vi "UMLEditor Main.vi"(1 "StartProject":string, 3 "StartTarget":string) -> ()   [LabVIEW 2020] (continued)
        n1589 = property class="Project"(reference=w4295) -> (reference out=w4292:refnum<vi>, error out=w4293:errorcluster, "Path"=w4291:path)  [unwired: 1 in]
        n1590 = call <resource>:"GetRelativePathOption.vi"() -> ("UseProjectFolderAsBasePath"=w4294:bool)  [unwired: 1 in, 18 out]
        n1591 = Strip Path(path=w4291) -> (stripped path=w4288:path)  [unwired: 1 out]
        n1592 = Close Reference(reference=w4292, error in (no error)=w4293) -> (error out=w4287:errorcluster)
        n1593 = call <resource>:"File_ApplicationPaths.vi"("PathName"=UMLEditor_StoredPathes."LastSearchPath" ("UMLPathes"), "Path In"=w4288, "Method (Get Path)"=File_StoredPathesActions."Set Path") -> ()  [unwired: 1 in, 16 out]
        n1594 = case shown="True" w4294 {
          tunnel: w4288 -> [_ w4305]
          tunnel: w4287 -> [_ _]
          frame False {
          }
          frame True {
            n1595 = call <resource>:"File_ApplicationPaths.vi"("PathName"=UMLEditor_StoredPathes."ClassBasePath" ("UMLPathes"), "Path In"=w4305, "Method (Get Path)"=File_StoredPathesActions."Set Path") -> ()  [unwired: 1 in, 16 out]
          }
        }
      }
      frame "ClassReversedEngineering".."StateReversedEngineering" {
        n1596 = case shown="\"ClassReversedEngineering\", Default" w4310 {
          tunnel: w4317 -> [w4331 w4367 w4387]
          tunnel: [w4320 w4366 w4382] -> w4315
          tunnel: [w4323 w4365 w4387] -> w4314
          tunnel: [w4319 w4364 w4381] -> w4312
          tunnel: w4309 -> [w4318 w4361 w4383]
          tunnel: [w4318 w4362 w4383] -> w4308
          frame "StateReversedEngineering" {
            (unwired) T49."existing file" ("select mode (2)")
            n1597 = Unbundle By Name(w4318) -> ("grid"=w4321:refnum<class "Grid.lvclass">, "graphics"=w4322:refnum<class "Graphics.lvclass">)
            n1598 = File Dialog(4:"VIs" ("pattern label"), 6:"*.vi" ("pattern"), 7:"Select VI(containing a state machine) for analysing" ("prompt")) -> (1:w4327:bool, 3:w4326:path)  [unwired: 1 in, 5 out]
            n1599 = Bundle By Name(cluster=T29 {"VI-Path"=path "", "ShowOption"=enum."Show Relative Path"} ("StateDiagramData"), "VI-Path"=w4326) -> (w4324:T29)
            n1600 = case shown="False" w4327 {
              selector: w4327 -> [_ w4348]
              tunnel: w4331 -> [w4342 w4347]
              tunnel: w4324 -> [w4341 _]
              tunnel: [w4334 w4347] -> w4323
              tunnel: w4322 -> [w4338 _]
              tunnel: w4321 -> [w4337 _]
              tunnel: [w4333 w4348] -> w4320
              tunnel: [w4332 _] -> w4319
              frame False {
                n1601 = call <resource>:"StateDiagramGraph_Create.vi"("StateDiagramData"=w4341, "error in (no error)"=w4342) -> ("reference out"=w4340:refnum<class "StateDiagramGraph.lvclass">, "error out"=w4339:errorcluster)  [unwired: 1 in, 15 out]
                n1602 = call-dynamic "HandleRightClickMenuOption.vi"("reference"=w4340, "MenuOption"="Create New Diagram", "graphics"=w4338, "grid"=w4337, "error in (no error)"=w4339) -> ("reference out"=w4332:refnum<class "StateDiagramGraph.lvclass">, "Cancel"=w4333:bool, "error out"=w4335:errorcluster)  [unwired: 12 in]
                n1603 = case shown="False" w4333 {
                  tunnel: w4332 -> [_ w4346]
                  tunnel: w4335 -> [w4343 w4345]
                  tunnel: [w4343 w4344] -> w4334
                  frame False {
                  }
                  frame True {
                    n1604 = call-dynamic "Destroy.vi"("reference"=w4346, "error in (no error)"=w4345) -> ("error out"=w4344:errorcluster)  [unwired: 17 in]
                  }
                }
              }
              frame True {
              }
            }
          }
          frame "ClassReversedEngineering", Default {
            n1605 = Unbundle By Name(w4361) -> ("XMI_Import"=w4349:bool, "Action"=w4358:string)
            n1606 = String To Path(string=w4358) -> (path=w4351:path)
            n1607 = File/Directory Info(path=w4351) -> (size=w4357:i64)  [unwired: 1 in, 6 out]
            n1608 = call <vilib>:"Librarian Get Info.vi"("path"=w4351) -> ("file information"=w4355:T55)  [unwired: 1 in, 9 out]
            n1609 = Unbundle By Name(w4355) -> ("size"=w4354:i32)
            n1610 = Greater Than 0?(x=w4357) -> (x > 0?=w4356:bool)
            n1611 = Greater Than 0?(x=w4354) -> (x > 0?=w4353:bool)
            n1612 = Equal?(x=w4358, y="WholeProject") -> (x = y?=w4359:bool)
            n1613 = Or(x=w4356, y=w4353) -> (x .or. y?=w4352:bool)
            n1614 = case shown="False" w4352 {
              tunnel: w4367 -> [w4373 w4379]
              tunnel: [w4372 w4378] -> w4366
              tunnel: [w4371 w4377] -> w4365
              tunnel: [w4370 w4376] -> w4364
              tunnel: w4359 -> [w4369 _]
              tunnel: w4351 -> [_ w4375]
              tunnel: w4349 -> [w4368 w4374]
              frame False {
                n1615 = call <resource>:"UMLEditor reversedEngineering.vi"("AddProjectClasses"=w4369, "XMI Import"=w4368, "error in (no error)"=w4373) -> ("cancel"=w4372:bool, "newCLassDiagram"=w4370:refnum<class "Graph.lvclass">, "error out"=w4371:errorcluster)  [unwired: 1 in, 13 out]
              }
              frame True {
                n1616 = call <resource>:"UMLEditor reversedEngineering.vi"("ClassToAnalyse/XMI File To Read"=w4375, "XMI Import"=w4374, "error in (no error)"=w4379) -> ("cancel"=w4378:bool, "newCLassDiagram"=w4376:refnum<class "Graph.lvclass">, "error out"=w4377:errorcluster)  [unwired: 1 in, 13 out]
              }
            }
            n1617 = Bundle By Name(cluster=w4361, "Action"="", "XMI_Import"=FALSE) -> (w4362:T5)
          }
          frame "PlugInReverseEngineering" {
            n1618 = call <resource>:"File_ApplicationPaths.vi"("PathName"=UMLEditor_StoredPathes."RevPlugInPath" ("UMLPathes")) -> ("Path Out"=w4384:path)  [unwired: 3 in, 15 out]
            n1619 = Open VI Reference(type specifier VI Refnum (for type only)=refnum<vi> refnum, vi path=w4384, error in (no error)=w4387) -> (vi reference=w4391:refnum<vi>, error out=w4390:errorcluster)  [unwired: 3 out]
            n1620 = call-by-ref "?"(reference=w4391, error in=w4390) -> (reference out=w4389:refnum<vi>, error out=w4388:errorcluster, "reference"=w4381:refnum<class "Graph.lvclass">, "cancelled"=w4382:bool, "diagramType"=w4380:T56)  [unwired: 8 in, 1 out]
            n1621 = Close Reference(reference=w4389, error in (no error)=w4388) -> (error out=w4386:errorcluster)
            n1622 = Format Into String(w4380) -> ()  [unwired: 3 in, 2 out]
            n1623 = call <vilib>:"Simple Error Handler.vi"("error in (no error)"=w4386) -> ()  [unwired: 1 in, 8 out]
          }
        }
        n1624 = case shown="False" w4315 {
          tunnel: w4314 -> [w4406 w4430]
          tunnel: [w4412 w4430] -> w4316
          tunnel: [w4410 w4428] -> w4313
          tunnel: w4312 -> [w4407 _]
          tunnel: [UMLEditor_statesType."Repaint" ("state") UMLEditor_statesType."Idle" ("state")] -> w4311
          tunnel: w4308 -> [w4396 w4428]
          frame False {
            n1625 = Unbundle By Name(w4396) -> ("diagrams"=w4422:T8[])
            n1626 = Unbundle By Name(w4396) -> ("grid"=w4403:refnum<class "Grid.lvclass">, "graphics"=w4404:refnum<class "Graphics.lvclass">)
            n1627 = for {
              tunnel: w4422 -> [w4427] mode=indexing
              tunnel: "Untitled %d" -> [w4425]
              tunnel: [w4424] -> w4420 mode=indexing
              n1628 = Unbundle By Name(w4427) -> ("name"=w4426:string)
              n1629 = Scan From String(format string=w4425, input string=w4426) -> (output 1=w4424:i32)  [unwired: 2 in, 4 out]
            }
            n1630 = Array Max & Min(array=w4420) -> (max value=w4419:i32)  [unwired: 3 out]
            n1631 = call-dynamic "draw.vi"("reference"=w4407, "graphics"=w4404, "grid"=w4403, "error in (no error)"=w4406, "SelectedNodes"=refnum<class "AbstractNode.lvclass">[] [], "HideOverLays(False)"=FALSE) -> ("NodesBounds"=w4402:T10, "error out"=w4405:errorcluster)  [unwired: 10 in, 2 out]
            n1632 = Increment(x=w4419) -> (x+1=w4417:i32)
            n1633 = Bundle By Name(cluster=w4396, "NodesBounds"=w4402) -> (w4399:T5)
            n1634 = Format Into String(format string="Untitled %d", w4417) -> (resulting string=w4408:string)  [unwired: 2 in, 1 out]
            n1635 = property on="Diagram" class="Ring (strict)"("Tip Strip"=w4408) -> ()  [unwired: 2 in, 2 out]
            n1636 = Unbundle By Name(w4399) -> ("menu"=w4398:refnum<k9>)
            n1637 = call <resource>:"UMLEditor addDiagram.vi"("graph"=w4407, "name"=w4408, "saveDir"=path "", "unsaved(False)"=TRUE, "error in (no error)"=w4405, "localVariablesIn"=w4399) -> ("localVariablesOut"=w4397:T5, "error out"=w4415:errorcluster)  [unwired: 1 in, 11 out]
            n1638 = property on="GraphButtons" class="RadioBtnsControl (strict)"("Disabled"=u8 0) -> ()  [unwired: 2 in, 2 out]
            n1639 = call <resource>:"UMLEditor menuUpdates.vi"("menu"=w4398, "menuAction"=UMLEditor_MenuActionType."EnableSave", "error in (no error)"=w4415) -> ("error out"=w4411:errorcluster)  [unwired: 3 in, 13 out]
            n1640 = local write "Diagram"(0) -> ()
            n1641 = property on="Picture" class="Pict"("Visible"=TRUE) -> ()  [unwired: 2 in, 2 out]
            n1642 = call <resource>:"UMLEditor setDiagramInfo.vi"("error in (no error)"=w4411, "localVariablesIn"=w4397, "action"=enum16{"Name/Dir", "Unsaved", "Saved"}."Unsaved") -> ("localVariablesOut"=w4410:T5, "error out"=w4412:errorcluster)  [unwired: 2 in, 13 out]
          }
          frame True {
          }
        }
      }
      frame "PanAndRepaint" {
        n1643 = Unbundle By Name(w4450) -> ("graphics"=w4449:refnum<class "Graphics.lvclass">, "SelectedNodes"=w4448:refnum<class "AbstractNode.lvclass">[])
        n1644 = Index Array(array=w4448) -> (element=w4447:refnum<class "AbstractNode.lvclass">)  [unwired: 1 in]
        n1645 = To More Specific Class(target class=refnum<class "RectangularNode.lvclass"> refnum ("reference"), reference=w4447, error in=w4445) -> (specific class reference=w4444:refnum<class "RectangularNode.lvclass">, error out=w4443:errorcluster)
        n1646 = call <resource>:"getScreenBounds.vi"("reference"=w4449) -> ("bounds"=w4438:T10)  [unwired: 1 in, 17 out]
        n1647 = call-dynamic "getBounds.vi"("reference"=w4444, "error in (no error)"=w4443) -> ("bounds"=w4432:T10, "error out"=w4434:errorcluster)  [unwired: 15 in, 1 out]
        n1648 = Unbundle By Name(w4438) -> ("width"=w4433:dbl, "height"=w4431:dbl)
        n1649 = property on="Picture" class="Pict"() -> ("Origin:Left"=w4440:i16, "Origin:Top"=w4439:i16)  [unwired: 2 in, 2 out]
        n1650 = Unbundle By Name(w4432) -> ("x"=w4442:dbl, "y"=w4441:dbl)
        n1651 = In Range and Coerce(upper limit=w4433, x=w4442, lower limit=w4440) -> (In Range?=w4437:bool)  [unwired: 1 out]
        n1652 = In Range and Coerce(upper limit=w4431, x=w4441, lower limit=w4439) -> (In Range?=w4436:bool)  [unwired: 1 out]
        n1653 = And(x=w4437, y=w4436) -> (x .and. y?=w4435:bool)
        n1654 = case shown="False" w4435 {
          tunnel: w4433 -> [w4465 _]
          tunnel: w4432 -> [w4463 _]
          tunnel: w4431 -> [w4458 _]
          frame False {
            w4452 = 0.0 ("y")
            n1655 = call <resource>:"Rectangel GetRectInfo.vi"("bounds"=w4463) -> ("centerX"=w4462:dbl, "centerY"=w4460:dbl)  [unwired: 14 in, 3 out]
            n1656 = Divide(x=w4465, y=2.0) -> (x/y=w4461:dbl)
            n1657 = Divide(x=w4458, y=2.0) -> (x/y=w4457:dbl)
            n1658 = Subtract(x=w4462, y=w4461) -> (x-y=w4456:dbl)
            n1659 = Subtract(x=w4460, y=w4457) -> (x-y=w4454:dbl)
            n1660 = Max & Min(x=w4456, y=w4452) -> (max(x,y)=w4455:dbl)  [unwired: 1 out]
            n1661 = Max & Min(x=w4454, y=w4452) -> (max(x,y)=w4453:dbl)  [unwired: 1 out]
            n1662 = property on="Picture" class="Pict"("Origin:Left"=w4455, "Origin:Top"=w4453) -> ()  [unwired: 2 in, 2 out]
          }
          frame True {
          }
        }
      }
      frame "Repaint" {
        n1663 = Unbundle By Name(w4474) -> ("selected"=w4486:T7)
        n1664 = call <resource>:"UMLEditor getDiagramInfo.vi"("localVariables"=w4474, "error in (no error)"=w4484) -> ("graph"=w4471:refnum<class "Graph.lvclass">, "diagramType"=w4478:T27, "error out"=w4479:errorcluster)  [unwired: 15 out]
        n1665 = case shown="\"Node\"" w4486 {
          tunnel: [w4499 UMLEditor_MenuActionType."enablePropDel" ("menuAction") UMLEditor_MenuActionType."enablePropDel" ("menuAction")] -> w4485
          tunnel: w4478 -> [w4498 _ _]
          tunnel: [UMLEditor_MenuActionType."DisableCopy" ("menuAction") UMLEditor_MenuActionType."EnableCopy" ("menuAction") UMLEditor_MenuActionType."DisableCopy" ("menuAction")] -> w4468
          frame "None", Default {
            n1666 = case shown="Default" w4498 {
              tunnel: [UMLEditor_MenuActionType."enablePropDisDel" ("menuAction") UMLEditor_MenuActionType."disablePropDel" ("menuAction")] -> w4499
              frame "StateDiagramGraph" {
              }
              frame Default {
              }
            }
          }
          frame "Node" {
          }
          frame "Edge" {
          }
        }
        n1667 = Unbundle By Name(w4474) -> ("menu"=w4469:refnum<k9>)
        n1668 = Empty String/Path?(string/path=w4478) -> (empty?=w4483:bool)
        n1669 = call <resource>:"UMLEditor ToolsMenuUpdates.vi"("menu"=w4469, "Graph"=w4471, "error in (no error)"=w4479) -> ("error out"=w4467:errorcluster)  [unwired: 3 in, 13 out]
        n1670 = disable-structure shown="Enabled" {
          disable-tunnel: w4469 -> [w4495 _]
          disable-tunnel: w4468 -> [w4494 _]
          disable-tunnel: w4467 -> [w4493 w4496]
          disable-tunnel: [w4492 w4496] -> w4466
          frame Disabled {
            n1671 = call <resource>:"UMLEditor menuUpdates.vi"("menu"=w4495, "menuAction"=w4494, "error in (no error)"=w4493) -> ("error out"=w4492:errorcluster)  [unwired: 3 in, 13 out]
          }
          frame Enabled {
          }
        }
        n1672 = call <resource>:"UMLEditor menuUpdates.vi"("menu"=w4469, "menuAction"=w4485, "error in (no error)"=w4466) -> ("error out"=w4487:errorcluster)  [unwired: 3 in, 13 out]
        n1673 = call <resource>:"UMLEditor updateDiagramsInfo.vi"("localVariables"=w4474, "error in (no error)"=w4487) -> ("diagramNames"=w4491:string[], "index"=w4477:i32, "currentIsUnsaved"=w4473:bool, "notSavedBefore"=w4488:bool, "error out"=w4472:errorcluster)  [unwired: 13 out]
        n1674 = property on="Diagram" class="Ring (strict)"() -> ("Strings []"=w4490:string[])  [unwired: 2 in, 2 out]
        n1675 = feedback #6() -> (w4470:i32)  [unwired: 1 in]
        n1676 = feedback-in #6(w4477) -> ()
        n1677 = Not Equal?(x=w4470, y=w4477) -> (x != y?=w4475:bool)
        n1678 = Not Equal?(x=w4491, y=w4490) -> (x != y?=w4489:bool)
        n1679 = Or(x=w4475, y=w4489) -> (x .or. y?=w4476:bool)
        n1680 = case shown="True" w4476 {
          tunnel: w4491 -> [_ w4510]
          tunnel: w4477 -> [_ w4508]
          tunnel: w4473 -> [_ w4507]
          tunnel: w4488 -> [_ w4509]
          tunnel: w4469 -> [_ w4506]
          frame False {
          }
          frame True {
            (unwired) u16 0 items=["Class diagram: Untitled 1 *"] ("Diagram")
            n1681 = Compound Arithmetic op=AND(w4507, invert w4509) -> ()  [unwired: 1 out]
            n1682 = property on="Diagram" class="Ring (strict)"("Strings []"=w4510) -> ()  [unwired: 2 in, 2 out]
            n1683 = local write "Diagram"(w4508) -> ()
            n1684 = case shown="False" w4507 {
              tunnel: w4506 -> [w4511 w4513]
              frame True {
                n1685 = call <resource>:"UMLEditor menuUpdates.vi"("menu"=w4511, "menuAction"=UMLEditor_MenuActionType."EnableSave") -> ()  [unwired: 4 in, 14 out]
              }
              frame False {
                n1686 = call <resource>:"UMLEditor menuUpdates.vi"("menu"=w4513, "menuAction"=UMLEditor_MenuActionType."DiableSave") -> ()  [unwired: 4 in, 14 out]
              }
            }
          }
        }
        n1687 = Select(t=UMLEditor_statesType."Idle", s=w4483, f=UMLEditor_statesType."PaintComponent" ("state")) -> (s? t:f=w4481:T6)
      }
      frame "PaintComponent" {
        n1688 = Unbundle By Name(w4528) -> ("menu"=w4527:refnum<k9>)
        n1689 = Unbundle By Name(w4528) -> ("selected"=w4537:T7, "selectedEdge"=w4547:refnum<class "AbstractEdge.lvclass">, "SelectedNodes"=w4522:refnum<class "AbstractNode.lvclass">[], "ObjectHotspots"=w4521:T15[], "NodesBounds"=w4535:T10)
        n1690 = Unbundle By Name(w4528) -> ("newSelected"=w4544:bool, "zoom"=w4551:dbl, "grid"=w4545:refnum<class "Grid.lvclass">, "offset"=w4538:T9, "graphics"=w4541:refnum<class "Graphics.lvclass">, "hideGrid"=w4550:bool)  [unwired: 1 out]
        n1691 = Unbundle By Name(w4528) -> ("butDwn"=w4531:bool)
        n1692 = Unbundle By Name(w4528) -> ("ResizePanelInProgress"=w4532:bool)
        n1693 = call <resource>:"UMLEditor getDiagramInfo.vi"("localVariables"=w4528, "error in (no error)"=w4549) -> ("graph"=w4529:refnum<class "Graph.lvclass">, "error out"=w4539:errorcluster)  [unwired: 16 out]
        n1694 = case shown="False" w4544 {
          tunnel: w4551 -> [w4567 _]
          tunnel: w4550 -> [w4568 _]
          tunnel: w4529 -> [w4583 w4615]
          tunnel: [w4582 w4615] -> w4548
          tunnel: [w4581 w4616] -> w4530
          tunnel: w4539 -> [w4580 w4616]
          tunnel: w4541 -> [w4579 _]
          tunnel: w4545 -> [w4578 _]
          tunnel: w4540 -> [_ _]
          tunnel: w4538 -> [w4577 _]
          tunnel: [w4570 w4614] -> w4536
          tunnel: w4535 -> [w4571 w4614]
          tunnel: w4522 -> [w4563 _]
          tunnel: [w4562 w4611] -> w4519
          tunnel: w4521 -> [_ w4613]
          frame False {
            n1695 = call <resource>:"resetPicture.vi"("reference"=w4579, "error in (no error)"=w4580) -> ("reference out"=w4576:refnum<class "Graphics.lvclass">, "error out"=w4575:errorcluster)  [unwired: 16 out]
            n1696 = call <resource>:"getScreenBounds.vi"("reference"=w4576, "error in (no error)"=w4575) -> ("reference out"=w4574:refnum<class "Graphics.lvclass">, "bounds"=w4572:T10, "ZoomChanged"=w4564:bool, "error out"=w4573:errorcluster)  [unwired: 14 out]
            n1697 = Less?(x=w4567, y=0.5) -> (x < y?=w4565:bool)
            n1698 = Or(x=w4565, y=w4568) -> (x .or. y?=w4569:bool)
            n1699 = case shown="False" w4569 {
              tunnel: w4578 -> [w4609 _]
              tunnel: w4567 -> [_ _]
              tunnel: [w4608 w4610] -> w4584
              tunnel: w4577 -> [_ _]
              tunnel: w4574 -> [w4607 _]
              tunnel: w4573 -> [w4606 w4610]
              tunnel: w4572 -> [w4601 _]
              tunnel: w4571 -> [w4605 _]
              tunnel: w4564 -> [w4590 _]
              frame False {
                w4585 = 500
                w4603 = 50
                w4600 = 0.0 ("x")
                n1700 = Unbundle By Name(w4605) -> ("width"=w4604:dbl, "height"=w4602:dbl)
                n1701 = Unbundle By Name(w4601) -> ("width"=w4599:dbl, "height"=w4598:dbl)
                n1702 = property on="Picture" class="Pict"() -> ("Origin:Left"=w4593:i16, "Origin:Top"=w4592:i16)  [unwired: 2 in, 2 out]
                n1703 = Add(x=w4603, y=w4602) -> (x+y=w4594:dbl)
                n1704 = Add(x=w4603, y=w4604) -> (x+y=w4597:dbl)
                n1705 = Add(x=w4593, y=w4599) -> (x+y=w4596:dbl)
                n1706 = Add(x=w4592, y=w4598) -> (x+y=w4595:dbl)
                n1707 = Max & Min(x=w4597, y=w4596) -> (max(x,y)=w4589:dbl)  [unwired: 1 out]
                n1708 = Max & Min(x=w4594, y=w4595) -> (max(x,y)=w4587:dbl)  [unwired: 1 out]
                n1709 = Add(x=w4585, y=w4587) -> (x+y=w4586:dbl)
                n1710 = Add(x=w4585, y=w4589) -> (x+y=w4588:dbl)
                n1711 = Bundle(cluster=w4601, "x"=w4600, "y"=w4600, "width"=w4588, "height"=w4586) -> (w4591:T10)
                n1712 = call-dynamic "draw.vi"("reference"=w4609, "graphics"=w4607, "bounds"=w4591, "ForceRedrawGrid"=w4590, "error in (no error)"=w4606) -> ("error out"=w4608:errorcluster)  [unwired: 13 in, 1 out]
              }
              frame True {
              }
            }
            n1713 = call-dynamic "draw.vi"("reference"=w4583, "graphics"=w4579, "grid"=w4578, "error in (no error)"=w4584, "SelectedNodes"=w4563, "HideOverLays(False)"=FALSE) -> ("reference out"=w4582:refnum<class "Graph.lvclass">, "NodesBounds"=w4570:T10, "HotSpots"=w4562:T15[], "error out"=w4581:errorcluster)  [unwired: 10 in]
          }
          frame True {
            n1714 = for {
              tunnel: w4613 -> [w4618] mode=indexing
              shift-right: [w4617] -> w4611
              shift-left: T15[] [] -> [w4619]
              n1715 = Unbundle By Name(w4618) -> ("Function"=w4620:T16)
              n1716 = case shown="\"Expand\", \"Collaps\"" w4620 {
                tunnel: w4619 -> [w4621 w4624]
                tunnel: w4618 -> [_ w4623]
                tunnel: [w4621 w4622] -> w4617
                frame Default {
                }
                frame "Expand", "Collaps" {
                  n1717 = Build Array (concatenate)(w4624, w4623) -> (w4622:T15[])
                }
              }
            }
          }
        }
        n1718 = Compound Arithmetic op=AND(invert w4531, invert w4532) -> (w4526:bool)
        n1719 = call <resource>:"UMLEditor_GraphMemory.vi"("GraphIn"=w4529) -> ()  [unwired: 1 in, 18 out]
        n1720 = call <resource>:"updateScreen.vi"("reference"=w4541, "error in (no error)"=w4530) -> ("reference out"=w4525:refnum<class "Graphics.lvclass">, "picture"=w4515:picture, "error out"=w4542:errorcluster)  [unwired: 15 out]
        n1721 = case shown="True" w4526 {
          tunnel: w4530 -> [w4555 w4560]
          tunnel: [w4555 w4559] -> _
          tunnel: w4529 -> [_ w4558]
          tunnel: w4527 -> [_ w4556]
          frame False {
          }
          frame True {
            n1722 = call <resource>:"UndoEngine.vi"("Reference In"=w4558, "Action"=enum16{"TakeSnapshot", "Undo", "Redo"}."TakeSnapshot", "error in (no error)"=w4560, "menu"=w4556) -> ("error out"=w4559:errorcluster)  [unwired: 4 in, 11 out]
          }
        }
        n1723 = case shown="\"Edge\"" w4537 {
          tunnel: [w4628 w4637 w4676] -> w4518
          tunnel: w4548 -> [_ w4640 w4682]
          tunnel: w4542 -> [w4628 w4639 w4681]
          tunnel: w4547 -> [_ w4633 _]
          tunnel: [TRUE w4632 w4678] -> w4533
          tunnel: w4541 -> [_ w4636 w4675]
          tunnel: w4522 -> [_ _ w4680]
          tunnel: w4525 -> [_ w4631 w4672]
          tunnel: [w4626 w4630 w4673] -> w4520
          tunnel: w4519 -> [w4626 w4630 w4671]
          tunnel: w4515 -> [w4625 w4629 w4668]
          frame "None", Default {
            n1724 = local write "Picture"(w4625) -> ()
          }
          frame "Edge" {
            n1725 = call-dynamic "getEdges.vi"("reference"=w4640, "error in (no error)"=w4639) -> ("edges"=w4638:refnum<class "AbstractEdge.lvclass">[], "error out"=w4635:errorcluster)  [unwired: 15 in, 1 out]
            n1726 = Search 1D Array(1D array=w4638, element=w4633) -> (index of element=w4634:i32)  [unwired: 1 in]
            n1727 = case shown="0, Default" w4634 {
              tunnel: [w4655 w4667] -> w4637
              tunnel: w4636 -> [w4654 _]
              tunnel: w4635 -> [w4653 w4667]
              tunnel: w4633 -> [w4643 _]
              tunnel: w4631 -> [w4641 _]
              tunnel: w4629 -> [_ w4666]
              frame 0, Default {
                n1728 = To More Specific Class(target class=refnum<class "GeneralPathEdge.lvclass"> refnum ("reference out"), reference=w4643) -> (specific class reference=w4642:refnum<class "GeneralPathEdge.lvclass">, error out=w4644:errorcluster)  [unwired: 1 in]
                n1729 = case shown="No Error" w4644 {
                  tunnel: w4653 -> [w4660 w4665]
                  tunnel: [w4656 w4664] -> w4652
                  tunnel: [w4657 w4663] -> w4651
                  tunnel: [w4658 w4662] -> w4649
                  tunnel: w4643 -> [_ w4661]
                  tunnel: w4642 -> [w4659 _]
                  frame No Error {
                    n1730 = call-dynamic "getPath.vi"("reference"=w4659, "error in (no error)"=w4660) -> ("reference out"=w4658:refnum<class "GeneralPathEdge.lvclass">, "points"=w4656:T9[], "error out"=w4657:errorcluster)  [unwired: 15 in]
                  }
                  frame Error {
                    n1731 = call-dynamic "getConnectionPoints.vi"("reference"=w4661, "error in (no error)"=w4665) -> ("reference out"=w4662:refnum<class "AbstractEdge.lvclass">, "connectionPoints"=w4664:T9[], "error out"=w4663:errorcluster)  [unwired: 15 in]
                  }
                }
                n1732 = call-dynamic "GetTextPositions.vi"("reference"=w4649, "GraphicsRef"=w4641, "error in (no error)"=w4651) -> ("connectionPoints"=w4647:T9[], "error out"=w4650:errorcluster)  [unwired: 14 in, 1 out]
                n1733 = Build Array (concatenate)(w4652, w4647) -> (w4648:T9[])
                n1734 = call <resource>:"UMLEditor drawGrabbers.vi"("graphics"=w4654, "points"=w4648, "error in (no error)"=w4650) -> ("picture"=w4646:picture, "error out"=w4655:errorcluster)  [unwired: 15 out]
                n1735 = local write "Picture"(w4646) -> ()
              }
              frame -1 {
                "Picture" <- w4666
              }
            }
            n1736 = Less Than 0?(x=w4634) -> (x < 0?=w4632:bool)
          }
          frame "Node" {
            n1737 = Array Size(array=w4680) -> (size(s)=w4679:i32)
            n1738 = for {
              tunnel: w4682 -> [w4700]
              tunnel: w4680 -> [w4696] mode=indexing
              shift-right: [w4695] -> w4677
              shift-left: w4681 -> [_]
              shift-right: [w4693] -> w4670
              shift-left: T9[] [] -> [w4694]
              shift-right: [w4692] -> w4673
              shift-left: w4671 -> [w4691]
              tunnel: w4672 -> [w4690]
              n1739 = call-dynamic "getNodes.vi"("reference"=w4700) -> ("nodes"=w4699:refnum<class "AbstractNode.lvclass">[], "error out"=w4698:errorcluster)  [unwired: 16 in, 1 out]
              n1740 = Search 1D Array(1D array=w4699, element=w4696) -> (index of element=w4697:i32)  [unwired: 1 in]
              n1741 = case shown="0, Default" w4697 {
                tunnel: [w4701 w4712] -> w4695
                tunnel: w4698 -> [w4708 w4712]
                tunnel: w4696 -> [w4703 _]
                tunnel: w4694 -> [w4709 w4711]
                tunnel: [w4707 w4711] -> w4693
                tunnel: [w4706 w4710] -> w4692
                tunnel: w4691 -> [w4705 w4710]
                tunnel: w4690 -> [_ _]
                frame 0, Default {
                  n1742 = call-dynamic "GetGrabberPositions.vi"("reference"=w4703, "error in (no error)"=w4708) -> ("GrabberPositions"=w4704:T9[], "HotSpots"=w4702:T15[], "error out"=w4701:errorcluster)  [unwired: 14 in, 1 out]
                  n1743 = Build Array (concatenate)(w4705, w4702) -> (w4706:T15[])
                  n1744 = Build Array (concatenate)(w4709, w4704) -> (w4707:T9[])
                }
                frame -1 {
                }
              }
            }
            n1745 = Less Or Equal To 0?(x=w4679) -> (x <= 0?=w4678:bool)
            n1746 = Empty Array?(array=w4670) -> (empty?=w4669:bool)
            n1747 = case shown="False" w4669 {
              tunnel: w4677 -> [w4687 w4689]
              tunnel: [w4686 w4689] -> w4676
              tunnel: w4675 -> [w4685 _]
              tunnel: w4670 -> [w4684 _]
              tunnel: w4668 -> [_ w4688]
              frame False {
                n1748 = call <resource>:"UMLEditor drawGrabbers.vi"("graphics"=w4685, "points"=w4684, "error in (no error)"=w4687) -> ("picture"=w4683:picture, "error out"=w4686:errorcluster)  [unwired: 15 out]
                n1749 = local write "Picture"(w4683) -> ()
              }
              frame True {
                n1750 = local write "Picture"(w4688) -> ()
              }
            }
          }
        }
        n1751 = Bundle By Name(cluster=w4528, "newSelected"=FALSE, "NodesBounds"=w4536) -> (w4534:T5)
        n1752 = case shown="True" w4533 {
          tunnel: [w4713 w4715] -> w4523
          tunnel: w4534 -> [w4713 w4716]
          frame False {
          }
          frame True {
            n1753 = Bundle By Name(cluster=w4716, "selected"=UMLEditor_tooltype."None" ("selcted")) -> (w4715:T5)
          }
        }
        n1754 = Tick Count (ms)() -> (millisecond timer value=w4516:u32)
        n1755 = case shown="True" w4517 {
          tunnel: w4518 -> [_ _]
          tunnel: w4516 -> [_ w4552]
          frame False {
          }
          frame True {
            n1756 = Tick Count (ms)() -> (millisecond timer value=w4554:u32)
            n1757 = Subtract(x=w4554, y=w4552) -> (x-y=→"Time":u32)
          }
        }
        n1758 = Bundle By Name(cluster=w4523, "ObjectHotspots"=w4520) -> (w4524:T5)
      }
      frame "AutoPlace" {
        n1759 = call <resource>:"ArrangeNodes Main.vi"("localVariablesOut"=w4719) -> ("Cancel"=w4717:bool)  [unwired: 1 in, 17 out]
        n1760 = case shown="False" w4717 {
          tunnel: w4721 -> [w4724 w4730]
          tunnel: [w4724 w4729] -> w4720
          tunnel: [w4723 w4726] -> w4718
          tunnel: w4719 -> [w4723 w4728]
          frame True {
          }
          frame False {
            n1761 = call <resource>:"UMLEditor setDiagramInfo.vi"("error in (no error)"=w4730, "localVariablesIn"=w4728, "action"=enum16{"Name/Dir", "Unsaved", "Saved"}."Unsaved") -> ("localVariablesOut"=w4727:T5, "error out"=w4729:errorcluster)  [unwired: 2 in, 13 out]
            n1762 = Bundle By Name(cluster=w4727, "modified"=TRUE) -> (w4726:T5)
          }
        }
      }
      frame "ExecuteCommand" {
        n1763 = Unbundle By Name(w4735) -> ("FlattenCommandSettings.Command"=w4743:T13, "FlattenCommandSettings.CommandData"=w4737:variant, "selected"=w4742:T7, "selectedEdge"=w4732:refnum<class "AbstractEdge.lvclass">, "SelectedNodes"=w4739:refnum<class "AbstractNode.lvclass">[])
        n1764 = Unbundle By Name(w4735) -> ("graphics"=w4734:refnum<class "Graphics.lvclass">, "grid"=w4733:refnum<class "Grid.lvclass">)
        n1765 = call <resource>:"UMLEditor getDiagramInfo.vi"("localVariables"=w4735, "error in (no error)"=w4741) -> ("graph"=w4736:refnum<class "Graph.lvclass">, "error out"=w4740:errorcluster)  [unwired: 16 out]
        n1766 = case shown="\"SyncCodeFromUML\"" w4743 {
          tunnel: [w4756 w4832 UMLEditor_statesType."Idle" ("state") UMLEditor_statesType."Idle" ("state") UMLEditor_statesType."CreateScript" ("state") UMLEditor_statesType."Idle" ("state") UMLEditor_statesType."Idle" ("state") w5042 UMLEditor_statesType."Idle" ("state")] -> w4745
          tunnel: w4740 -> [w4755 w4839 w4863 w4868 w4893 w4899 w4916 w5060 w5086]
          tunnel: [w4752 w4844 w4863 w4868 w4893 w4898 w4914 w5060 w5085] -> w4744
          tunnel: w4742 -> [w4754 w4837 _ _ _ _ _ _ _]
          tunnel: w4739 -> [w4753 w4835 _ _ _ _ _ w5061 w5083]
          tunnel: w4735 -> [w4751 w4843 w4865 w4881 w4891 w4908 w4921 w5041 w5088]
          tunnel: [w4750 w4842 w4865 w4881 w4891 w4908 w4921 w5040 w5088] -> w4738
          tunnel: w4736 -> [w4749 w4841 _ _ _ _ _ _ _]
          tunnel: w4737 -> [_ w4838 w4866 w4882 w4895 w4909 w4922 _ _]
          tunnel: w4735 -> [w4748 _ _ _ _ _ _ _ _]
          tunnel: w4736 -> [_ w4840 _ _ _ _ _ _ w5087]
          tunnel: w4734 -> [w4747 _ _ _ _ _ _ _ _]
          tunnel: w4733 -> [w4746 _ _ _ _ _ _ _ _]
          tunnel: w4732 -> [_ w4836 _ _ _ _ _ _ _]
          frame "SyncUmlFromCode", Default {
            n1767 = case shown="\"Node\"" w4754 {
              tunnel: [UMLEditor_statesType."Repaint" ("state") UMLEditor_statesType."Repaint" ("state")] -> w4756
              tunnel: w4755 -> [w4759 w4783]
              tunnel: w4753 -> [_ w4785]
              tunnel: [w4759 w4788] -> w4752
              tunnel: w4751 -> [w4757 w4787]
              tunnel: [w4757 w4786] -> w4750
              tunnel: w4749 -> [_ w4780]
              tunnel: w4748 -> [_ _]
              tunnel: w4747 -> [_ w4779]
              tunnel: w4746 -> [_ w4778]
              frame "None", Default {
              }
              frame "Node" {
                n1768 = Index Array(array=w4785) -> (element=w4762:refnum<class "AbstractNode.lvclass">)  [unwired: 1 in]
                n1769 = To More Specific Class(target class=refnum<class "ClassNode.lvclass"> refnum ("reference"), reference=w4762) -> (specific class reference=w4761:refnum<class "ClassNode.lvclass">)  [unwired: 1 in, 1 out]
                n1770 = call-dynamic "getClassInfo.vi"("reference"=w4761, "error in (no error)"=w4783) -> ("methods(string)"=w4766:string, "attributes(string)"=w4773:string, "reference out"=w4781:refnum<class "ClassNode.lvclass">, "className"=w4777:string, "ClassPath"=w4784:path, "error out"=w4782:errorcluster)  [unwired: 8 in, 4 out]
                n1771 = call <resource>:"ReversedEngineering SyncUmlFromCode.vi"("SyncAction"=ReversedEngineering_SyncUmlFromCodeActions."GetAll", "ClassPath"=w4784, "NodeRef"=w4781, "GraphRef"=w4780, "error in (no error)"=w4782, "ClassName(needed for lllbs)"=w4777, "graphics"=w4779, "grid"=w4778) -> ("ClassName"=w4764:string, "attributes"=w4774:string, "methods"=w4772:string, "error out"=w4793:errorcluster)  [unwired: 4 in, 4 out]
                n1772 = Empty String/Path?(string/path=w4764) -> (empty?=w4763:bool)
                n1773 = Empty String/Path?(string/path=w4766) -> (empty?=w4776:bool)
                n1774 = Empty String/Path?(string/path=w4773) -> (empty?=w4775:bool)
                n1775 = Equal?(x=w4774, y=w4773) -> (x = y?=w4770:bool)
                n1776 = Equal?(x=w4772, y=w4766) -> (x = y?=w4771:bool)
                n1777 = And(x=w4776, y=w4775) -> (x .and. y?=w4768:bool)
                n1778 = And(x=w4770, y=w4771) -> (x .and. y?=w4769:bool)
                n1779 = Or(x=w4769, y=w4768) -> (x .or. y?=w4767:bool)
                n1780 = case shown="True" w4767 {
                  tunnel: w4793 -> [w4804 w4805]
                  tunnel: [w4803 FALSE ("CancelOut")] -> w4792
                  tunnel: [w4802 w4805] -> w4791
                  tunnel: [w4801 w4807] -> w4790
                  tunnel: [w4800 w4806] -> w4789
                  tunnel: w4774 -> [w4799 w4807]
                  tunnel: w4773 -> [w4798 _]
                  tunnel: w4772 -> [w4797 w4806]
                  tunnel: w4766 -> [w4796 _]
                  frame False {
                    n1781 = call <resource>:"UMLEditor UpdateMethodsAttributesDialog.vi"("OldAttributesIn"=w4798, "OldMethodsIn"=w4796, "New Attributes"=w4799, "New Methods"=w4797, "error in (no error)"=w4804) -> ("AttributesOut"=w4801:string, "MethodsOut"=w4800:string, "CancelOut"=w4803:bool, "error out"=w4802:errorcluster)  [unwired: 11 out]
                  }
                  frame True {
                  }
                }
                n1782 = Or(x=w4763, y=w4792) -> (x .or. y?=w4765:bool)
                n1783 = case shown="False" w4765 {
                  tunnel: w4791 -> [w4811 w4829]
                  tunnel: w4781 -> [w4815 _]
                  tunnel: w4790 -> [w4817 _]
                  tunnel: w4789 -> [w4820 _]
                  tunnel: [w4818 w4829] -> w4788
                  tunnel: w4787 -> [w4822 w4828]
                  tunnel: [w4821 w4828] -> w4786
                  tunnel: w4780 -> [w4810 _]
                  tunnel: w4764 -> [w4813 _]
                  frame False {
                    n1784 = call-dynamic "ExternalSetParam.vi"("reference"=w4815, "setParameter"=ExternalSetTypes."Name", "string"=w4813, "error in (no error)"=w4811) -> ("reference out"=w4814:refnum<class "ClassNode.lvclass">, "error out"=w4812:errorcluster)  [unwired: 14 in]
                    n1785 = call-dynamic "ExternalSetParam.vi"("reference"=w4814, "setParameter"=ExternalSetTypes."Attributes", "string"=w4817, "error in (no error)"=w4812) -> ("reference out"=w4825:refnum<class "ClassNode.lvclass">, "error out"=w4826:errorcluster)  [unwired: 14 in]
                    n1786 = call-dynamic "ExternalSetParam.vi"("reference"=w4825, "setParameter"=ExternalSetTypes."Methods", "string"=w4820, "error in (no error)"=w4826) -> ("error out"=w4809:errorcluster)  [unwired: 14 in, 1 out]
                    n1787 = call <resource>:"UMLEditor setDiagramInfo.vi"("error in (no error)"=w4809, "localVariablesIn"=w4822, "action"=enum16{"Name/Dir", "Unsaved", "Saved"}."Unsaved") -> ("localVariablesOut"=w4821:T5, "error out"=w4819:errorcluster)  [unwired: 2 in, 13 out]
                    n1788 = call-dynamic "layout.vi"("reference"=w4810, "error in (no error)"=w4819) -> ("error out"=w4818:errorcluster)  [unwired: 16 in, 1 out]
                  }
                  frame True {
                  }
                }
              }
            }
          }
          frame "GraphExecute" {
            n1789 = call <vilib>:"Set Busy.vi"("error in (no error)"=w4839) -> ("error out"=w4831:errorcluster)  [unwired: 9 in, 1 out]
            n1790 = call-dynamic "ExecuteCommand.vi"("reference in"=w4840, "CommandData"=w4838, "toolType"=w4837, "selectedEdge"=w4836, "SelectedNodes"=w4835, "error in (no error)"=w4831) -> ("Cancelled"=w4833:bool, "error out"=w4834:errorcluster)  [unwired: 11 in, 1 out]
            n1791 = call <vilib>:"Unset Busy.vi"("error in (no error)"=w4834) -> ("error out"=w4830:errorcluster)  [unwired: 10 in]
            n1792 = case shown="False" w4833 {
              tunnel: w4830 -> [w4846 w4855]
              tunnel: [w4848 w4855] -> w4844
              tunnel: w4843 -> [w4851 w4854]
              tunnel: [w4850 w4854] -> w4842
              tunnel: w4841 -> [w4847 _]
              tunnel: [UMLEditor_statesType."Repaint" ("state") UMLEditor_statesType."Idle" ("state")] -> w4832
              frame False {
                n1793 = call <resource>:"UMLEditor setDiagramInfo.vi"("error in (no error)"=w4846, "localVariablesIn"=w4851, "action"=enum16{"Name/Dir", "Unsaved", "Saved"}."Unsaved") -> ("localVariablesOut"=w4850:T5, "error out"=w4849:errorcluster)  [unwired: 2 in, 13 out]
                n1794 = call-dynamic "layout.vi"("reference"=w4847, "error in (no error)"=w4849) -> ("error out"=w4848:errorcluster)  [unwired: 16 in, 1 out]
              }
              frame True {
              }
            }
          }
          frame "OpenClass" {
            w4857 = "Refresh"  # Message
            w4861 = "Open class"  # Message
            n1795 = Variant To Data(type=path "", Variant=w4866) -> (data=w4859:path)  [unwired: 1 in, 1 out]
            n1796 = Path To String(path=w4859) -> (string=w4860:string)
            n1797 = call <resource>:"UMLEditor SendMessageToWizard.vi"("MessageType"=w4861, "MessageData"=w4860, "error in (no error)"=w4863) -> ("error out"=w4856:errorcluster)  [unwired: 1 in, 15 out]
            n1798 = call <resource>:"UMLEditor SendMessageToWizard.vi"("MessageType"=w4857, "AllowErrorPopup(True)"=FALSE, "error in (no error)"=w4856) -> ()  [unwired: 1 in, 16 out]
          }
          frame "OpenClassAttribute" {
            n1799 = Variant To Data(error in=w4868, type=path "", Variant=w4882) -> (data=w4878:path, error out=w4877:errorcluster)
            n1800 = call <resource>:"CreateReaderFromClass.vi"("ClassPath/LvClassRef"=w4878, "error in"=w4877) -> ("ClassReader"=w4876:refnum<class "ClassReader.lvclass">, "error out"=w4875:errorcluster)  [unwired: 16 out]
            n1801 = call-dynamic "GetAttributes.vi"("ClassReader in"=w4876, "OnlyGetReference"=TRUE ("OnlyGetPath"), "error in (no error)"=w4875) -> ("ClassReader out"=w4873:refnum<class "ClassReader.lvclass">, "ObjectAttributeReference"=w4870:refnum<vi>, "error out"=w4872:errorcluster)  [unwired: 14 out]
            n1802 = call-dynamic <resource>:"CleanUp.vi"("reference in"=w4873, "error in (no error)"=w4872) -> ("error out"=w4871:errorcluster)  [unwired: 17 out]
            n1803 = Not A Number/Path/Refnum?(number/path/refnum=w4870) -> (NaN/Path/Refnum?=w4869:bool)
            n1804 = case shown="False" w4869 {
              tunnel: [w4886 w4890] -> w4867
              tunnel: w4871 -> [w4885 w4890]
              tunnel: w4870 -> [w4884 _]
              frame False {
                n1805 = property class="VI"(reference=w4884, error in=w4885, "Front Panel.Open"=TRUE ("Front Panel Window:Open")) -> (reference out=w4887:refnum<vi>, error out=w4888:errorcluster)
                n1806 = Close Reference(reference=w4887, error in (no error)=w4888) -> (error out=w4886:errorcluster)
              }
              frame True {
              }
            }
            n1807 = case shown="Error" w4867 {
              frame No Error {
              }
              frame Error {
                n1808 = One Button Dialog(message="The file was not possible to open with this version of LabVIEW") -> ()  [unwired: 1 in, 1 out]
              }
            }
          }
          frame "CreateClass" {
            n1809 = Variant To Data(type=path "", Variant=w4895) -> ()  [unwired: 1 in, 2 out]
          }
          frame "OpenFile" {
            n1810 = Variant To Data(type=path "", Variant=w4909) -> (data=w4905:path)  [unwired: 1 in, 1 out]
            n1811 = call <resource>:"CommonVIs_UmlOpenVIRef.vi"("error in"=w4899) -> ("error out"=w4898:errorcluster, "AppRefOut"=w4897:refnum<vi>)  [unwired: 3 in, 6 out]
            n1812 = Open VI Reference(application reference (local)=w4897, vi path=w4905, error in (no error)=w4898) -> (vi reference=w4904:refnum<vi>, error out=w4900:errorcluster)  [unwired: 3 out]
            n1813 = property class="VI"(reference=w4904, error in=w4900, "Front Panel Window:Open"=TRUE) -> (reference out=w4902:refnum<vi>, error out=w4901:errorcluster)
            n1814 = Close Reference(reference=w4902, error in (no error)=w4901) -> (error out=w4896:errorcluster)
            n1815 = case shown="Error" w4896 {
              frame No Error {
              }
              frame Error {
                n1816 = One Button Dialog(message="The file was not possible to open with this version of LabVIEW") -> ()  [unwired: 1 in, 1 out]
              }
            }
          }
          frame "LocateInProject" {
            n1817 = call <resource>:"CommonVIs_UmlOpenVIRef.vi"("error in"=w4916) -> ("error out"=w4918:errorcluster, "ProjectNameOut"=w4917:string, "AppRefOut"=w4911:refnum<vi>)  [unwired: 3 in, 5 out]
            n1818 = Variant To Data(type=path "", Variant=w4922) -> (data=w4912:path)  [unwired: 1 in, 1 out]
            n1819 = call <resource>:"GDSProject_GetProjects.vi"("GetProjectRefByName"=w4917, "error in (no error)"=w4918) -> ("Project Refnum"=w4915:refnum<vi>, "error out"=w4914:errorcluster)  [unwired: 1 in, 15 out]
            n1820 = call <vilib>:"Get File Extension.vi"("file"=w4912) -> ("lowercase file extension"=w4913:string)  [unwired: 6 in, 4 out]
            n1821 = case shown="\"lvlib\"" w4913 {
              tunnel: w4915 -> [_ w4929 w4956 w4998]
              tunnel: w4914 -> [_ w4928 w4953 w4995]
              tunnel: w4912 -> [_ w4924 w4954 w4996]
              tunnel: w4911 -> [_ w4923 w4955 w4997]
              frame "False", Default {
              }
              frame "ctl", "vi" {
                n1822 = Open VI Reference(application reference (local)=w4923, vi path=w4924, error in (no error)=w4928) -> (vi reference=w4925:refnum<vi>, error out=w4934:errorcluster)  [unwired: 3 in]
                n1823 = invoke class="Project" method="Proj Item From Ref"(reference=w4929, error in=w4934, "VI"=w4925) -> (reference out=w4926:refnum<vi>, error out=w4933:errorcluster, "ProjItemFromRef"=w4930:refnum<vi>)  [unwired: 1 in, 1 out]
                n1824 = Not A Number/Path/Refnum?(number/path/refnum=w4930) -> (NaN/Path/Refnum?=w4931:bool)
                n1825 = Close Reference(reference=w4925, error in (no error)=w4933) -> (error out=w4932:errorcluster)
                n1826 = case shown="False" w4931 {
                  tunnel: [w4935 w4948] -> w4927
                  tunnel: w4930 -> [w4940 _]
                  tunnel: w4926 -> [w4939 w4950]
                  tunnel: w4932 -> [w4938 w4949]
                  frame False {
                    w4943 = TRUE ("Select")
                    n1827 = invoke class="Project" method="Open Window"(reference=w4939, error in=w4938) -> (error out=w4941:errorcluster)  [unwired: 1 in, 2 out]
                    n1828 = invoke class="ProjectItem" method="Make Item Visible in Tree"(reference=w4940, error in=w4941) -> (reference out=w4944:refnum<vi>, error out=w4942:errorcluster)  [unwired: 1 in, 1 out]
                    n1829 = invoke class="ProjectItem" method="SelectItem"(reference=w4944, error in=w4942, "Select"=w4943, "ClearPreviousSelection"=w4943) -> (reference out=w4937:refnum<vi>, error out=w4936:errorcluster)  [unwired: 1 in, 3 out]
                    n1830 = Close Reference(reference=w4937, error in (no error)=w4936) -> (error out=w4935:errorcluster)
                  }
                  frame True {
                    n1831 = property class="Project"(reference=w4950, error in=w4949) -> (error out=w4948:errorcluster, "Name"=w4946:string)  [unwired: 1 out]
                    n1832 = Format Into String(format string="This item: %s couldn't be found in the project" ("message"), w4946) -> (resulting string=w4945:string)  [unwired: 2 in, 1 out]
                    n1833 = One Button Dialog(message=w4945) -> ()  [unwired: 1 in, 1 out]
                  }
                }
                n1834 = Close Reference(reference=w4926, error in (no error)=w4927) -> ()  [unwired: 1 out]
              }
              frame "lvclass" {
                n1835 = invoke class="App" method="LVClass.Open"(reference=w4955, error in=w4953, "Path"=w4954) -> (error out=w4952:errorcluster, "LVClass.Open"=w4951:refnum<vi>)  [unwired: 1 in, 2 out]
                n1836 = disable-structure shown="Enabled" {
                  disable-tunnel: w4956 -> [w4966 w4991]
                  disable-tunnel: w4952 -> [w4964 w4989]
                  disable-tunnel: w4951 -> [w4958 w4988]
                  frame Disabled {
                    n1837 = property class="LVClassLibrary"(reference=w4958, error in=w4964) -> (error out=w4963:errorcluster, "Member Data"=w4962:refnum<vi>)  [unwired: 1 out]
                    n1838 = invoke class="Project" method="Proj Item From Ref"(reference=w4966, error in=w4963, "VI"=w4962) -> (reference out=w4961:refnum<vi>, error out=w4960:errorcluster, "ProjItemFromRef"=w4967:refnum<vi>)  [unwired: 1 in, 1 out]
                    n1839 = Not A Number/Path/Refnum?(number/path/refnum=w4967) -> (NaN/Path/Refnum?=w4968:bool)
                    n1840 = Close Reference(reference=w4962, error in (no error)=w4960) -> (error out=w4959:errorcluster)
                    n1841 = Close Reference(reference=w4958, error in (no error)=w4959) -> (error out=w4957:errorcluster)
                    n1842 = case shown="False" w4968 {
                      tunnel: [w4969 w4982] -> w4965
                      tunnel: w4967 -> [w4974 _]
                      tunnel: w4961 -> [w4973 w4984]
                      tunnel: w4957 -> [w4972 w4983]
                      frame False {
                        w4977 = TRUE ("Select")
                        n1843 = invoke class="Project" method="Open Window"(reference=w4973, error in=w4972) -> (error out=w4975:errorcluster)  [unwired: 1 in, 2 out]
                        n1844 = invoke class="ProjectItem" method="Make Item Visible in Tree"(reference=w4974, error in=w4975) -> (reference out=w4978:refnum<vi>, error out=w4976:errorcluster)  [unwired: 1 in, 1 out]
                        n1845 = invoke class="ProjectItem" method="SelectItem"(reference=w4978, error in=w4976, "Select"=w4977, "ClearPreviousSelection"=w4977) -> (reference out=w4971:refnum<vi>, error out=w4970:errorcluster)  [unwired: 1 in, 3 out]
                        n1846 = Close Reference(reference=w4971, error in (no error)=w4970) -> (error out=w4969:errorcluster)
                      }
                      frame True {
                        n1847 = property class="Project"(reference=w4984, error in=w4983) -> (error out=w4982:errorcluster, "Name"=w4980:string)  [unwired: 1 out]
                        n1848 = Format Into String(format string="This item: %s couldn't be found in the project" ("message"), w4980) -> (resulting string=w4979:string)  [unwired: 2 in, 1 out]
                        n1849 = One Button Dialog(message=w4979) -> ()  [unwired: 1 in, 1 out]
                      }
                    }
                    n1850 = Close Reference(reference=w4961, error in (no error)=w4965) -> ()  [unwired: 1 out]
                  }
                  frame Enabled {
                    n1851 = invoke class="Project" method="Open Window"(reference=w4991, error in=w4989) -> (reference out=w4990:refnum<vi>, error out=w4987:errorcluster)  [unwired: 1 in, 1 out]
                    n1852 = invoke class="LVClassLibrary" method="HiliteInProjectWindow"(reference=w4988, error in=w4987) -> (reference out=w4986:refnum<vi>, error out=w4985:errorcluster)  [unwired: 1 in, 1 out]
                    n1853 = Close Reference(reference=w4986, error in (no error)=w4985) -> (error out=w4992:errorcluster)
                    n1854 = Close Reference(reference=w4990, error in (no error)=w4992) -> ()  [unwired: 1 out]
                  }
                }
              }
              frame "lvlib" {
                n1855 = invoke class="App" method="Library.Open"(reference=w4997, error in=w4995, "path"=w4996) -> (error out=w4994:errorcluster, "Open Library"=w4993:refnum<vi>)  [unwired: 1 in, 2 out]
                n1856 = disable-structure shown="Enabled" {
                  disable-tunnel: w4998 -> [w5008 w5033]
                  disable-tunnel: w4994 -> [w5006 w5031]
                  disable-tunnel: w4993 -> [w5000 w5030]
                  frame Disabled {
                    n1857 = property class="Library"(reference=w5000, error in=w5006) -> (error out=w5005:errorcluster, "Member Data"=w5004)  [unwired: 1 out]
                    n1858 = invoke class="Project" method="Proj Item From Ref"(reference=w5008, error in=w5005, "VI"=w5004) -> (reference out=w5003:refnum<vi>, error out=w5002:errorcluster, "ProjItemFromRef"=w5009:refnum<vi>)  [unwired: 1 in, 1 out]
                    n1859 = Not A Number/Path/Refnum?(number/path/refnum=w5009) -> (NaN/Path/Refnum?=w5010:bool)
                    n1860 = Close Reference(reference=w5004, error in (no error)=w5002) -> (error out=w5001:errorcluster)
                    n1861 = Close Reference(reference=w5000, error in (no error)=w5001) -> (error out=w4999:errorcluster)
                    n1862 = case shown="False" w5010 {
                      tunnel: [w5011 w5024] -> w5007
                      tunnel: w5009 -> [w5016 _]
                      tunnel: w5003 -> [w5015 w5026]
                      tunnel: w4999 -> [w5014 w5025]
                      frame False {
                        w5019 = TRUE ("Select")
                        n1863 = invoke class="Project" method="Open Window"(reference=w5015, error in=w5014) -> (error out=w5017:errorcluster)  [unwired: 1 in, 2 out]
                        n1864 = invoke class="ProjectItem" method="Make Item Visible in Tree"(reference=w5016, error in=w5017) -> (reference out=w5020:refnum<vi>, error out=w5018:errorcluster)  [unwired: 1 in, 1 out]
                        n1865 = invoke class="ProjectItem" method="SelectItem"(reference=w5020, error in=w5018, "Select"=w5019, "ClearPreviousSelection"=w5019) -> (reference out=w5013:refnum<vi>, error out=w5012:errorcluster)  [unwired: 1 in, 3 out]
                        n1866 = Close Reference(reference=w5013, error in (no error)=w5012) -> (error out=w5011:errorcluster)
                      }
                      frame True {
                        n1867 = property class="Project"(reference=w5026, error in=w5025) -> (error out=w5024:errorcluster, "Name"=w5022:string)  [unwired: 1 out]
                        n1868 = Format Into String(format string="This item: %s couldn't be found in the project" ("message"), w5022) -> (resulting string=w5021:string)  [unwired: 2 in, 1 out]
                        n1869 = One Button Dialog(message=w5021) -> ()  [unwired: 1 in, 1 out]
                      }
                    }
                    n1870 = Close Reference(reference=w5003, error in (no error)=w5007) -> ()  [unwired: 1 out]
                  }
                  frame Enabled {
                    n1871 = invoke class="Project" method="Open Window"(reference=w5033, error in=w5031) -> (reference out=w5032:refnum<vi>, error out=w5029:errorcluster)  [unwired: 1 in, 1 out]
                    n1872 = invoke class="Library" method="HiliteInProjectWindow"(reference=w5030, error in=w5029) -> (reference out=w5028:refnum<vi>, error out=w5027:errorcluster)  [unwired: 1 in, 1 out]
                    n1873 = Close Reference(reference=w5028, error in (no error)=w5027) -> (error out=w5034:errorcluster)
                    n1874 = Close Reference(reference=w5032, error in (no error)=w5034) -> ()  [unwired: 1 out]
                  }
                }
              }
            }
          }
          frame "CreateVI" {
            n1875 = Index Array(array=w5061) -> (element=w5035:refnum<class "AbstractNode.lvclass">)  [unwired: 1 in]
            n1876 = To More Specific Class(target class=refnum<class "ClassNode.lvclass"> refnum ("reference"), reference=w5035) -> (specific class reference=w5036:refnum<class "ClassNode.lvclass">)  [unwired: 1 in, 1 out]
            n1877 = call <resource>:"CommonVIs_UmlOpenVIRef.vi"() -> ("AppRefOut"=w5038:refnum<vi>)  [unwired: 4 in, 7 out]
            n1878 = call-dynamic "getClassInfo.vi"("reference"=w5036, "error in (no error)"=w5060) -> ("className"=w5058:string, "ClassPath"=w5039:path, "error out"=w5059:errorcluster)  [unwired: 8 in, 7 out]
            n1879 = call <resource>:"CommonVIs SterotypeStringParser.vi"("SterotypeStringIn"=w5058) -> ("StereoType"=w5055:T34, "Sterotype"=w5047:string)  [unwired: 17 out]
            n1880 = call <resource>:"File_ApplicationPaths.vi"("PathName"=UMLEditor_StoredPathes."ApplicationTemplatePath" ("UMLPathes")) -> ("Path Out"=w5052:path)  [unwired: 3 in, 15 out]
            n1881 = call <resource>:"File_ApplicationPaths.vi"("PathName"=UMLEditor_StoredPathes."ViTemplatePath" ("UMLPathes")) -> ("Path Out"=w5051:path)  [unwired: 3 in, 15 out]
            n1882 = Equal?(x=CommonVIs_StereoType."APPLICATION", y=w5055) -> (x = y?=w5053:bool)
            n1883 = Select(t=w5052, s=w5053, f=w5051) -> (s? t:f=w5046:path)
            n1884 = Empty String/Path?(string/path=w5046) -> (empty?=w5048:bool)
            n1885 = case shown="False" w5048 {
              tunnel: [w5070 w5075] -> w5066
              tunnel: [w5069 w5074] -> w5064
              tunnel: w5059 -> [w5068 w5073]
              tunnel: w5046 -> [_ w5072]
              tunnel: w5038 -> [w5067 w5071]
              frame True {
                n1886 = New VI(8:w5068, 11:w5067) -> (0:w5069:errorcluster, 3:w5070:refnum<vi>)  [unwired: 5 out]
              }
              frame False {
                n1887 = New VI(8:w5073, 10:w5072, 11:w5071) -> (0:w5074:errorcluster, 3:w5075:refnum<vi>)  [unwired: 4 out]
              }
            }
            n1888 = property class="VI"(reference=w5066, error in=w5064, "Front Panel Window:Open"=TRUE) -> (reference out=w5056:refnum<vi>, error out=w5057:errorcluster)
            n1889 = invoke class="VI" method="Save.Instrument"(reference=w5056, error in=w5057, "Path to saved file"=w5039) -> (reference out=w5045:refnum<vi>, error out=w5044:errorcluster)  [unwired: 3 in, 4 out]
            n1890 = Format Into String(format string="Error occurred when trying to create %s\nPath:%s\nTemplateFilePath:%s", w5047, w5039, w5046) -> (resulting string=w5049:string)  [unwired: 2 in, 1 out]
            n1891 = Close Reference(reference=w5045, error in (no error)=w5044) -> (error out=w5043:errorcluster)
            n1892 = case shown="No Error" w5043 {
              tunnel: w5049 -> [_ w5082]
              tunnel: [UMLEditor_statesType."ExecuteCommand" ("state") UMLEditor_statesType."Idle" ("state")] -> w5042
              tunnel: w5041 -> [w5077 w5080]
              tunnel: [w5078 w5080] -> w5040
              frame No Error {
                n1893 = Bundle By Name(cluster=w5077, "FlattenCommandSettings.Command"=UMLEditor_ExecuteCommandType."SyncCodeFromUML") -> (w5078:T5)
              }
              frame Error {
                n1894 = One Button Dialog(message=w5082) -> ()  [unwired: 2 out]
              }
            }
          }
          frame "SyncCodeFromUML" {
            n1895 = Index Array(array=w5083) -> (element=w5084:refnum<class "AbstractNode.lvclass">)  [unwired: 1 in]
            n1896 = call <resource>:"UMLEditor SyncCodeFromUml.vi"("error in"=w5086, "graph"=w5087, "selectedNode"=w5084) -> ("error out"=w5085:errorcluster)  [unwired: 1 in, 7 out]
          }
        }
      }
      frame "ApplyDesignPattern" {
